vi "Network Read.vi"(8 "error in (no error)":errorcluster, 9 "Status_Cluster_in":T1={"simTime"=0.0, "simFrame"=0.0, "Connection Status"=enum."Disconnected", "Connection Command"=enum."Disconnect", "Last Error"=0, "Case selection"=enum."Connecting"}, 10 "RDB References in":T7, 11 "Settings":T4={"UDP Receiver"=refnum, "UDP Sender"=refnum, "Valid Packet"=FALSE, "TCP"=refnum, "Network Settings"={"IP adress"="127.0.0.1", "RDB"={"Protocol"=enum."UDP", "Tx Port"=48270, "Rx Port"=10, "Buffer Size"=204800, "Timeout"=10}, "SCP"={"Protocol"=enum."TCP", "Tx Port"=48191, "Rx Port"=48191, "Buffer Size"=204800, "Timeout"=10}}, "vclient"=path "", "paeseHandle"=0, "builderHandle"=0}) -> (0 "error out":errorcluster, 1 "Status_Cluster_out":T1={"simTime"=0.0, "simFrame"=0.0, "Connection Status"=enum."Disconnected", "Connection Command"=enum."Disconnect", "Last Error"=0, "Case selection"=enum."Connecting"}, 2 "RDB References out":T7, 3 "Settings":T4={"UDP Receiver"=refnum, "UDP Sender"=refnum, "Valid Packet"=FALSE, "TCP"=refnum, "Network Settings"={"IP adress"="127.0.0.1", "RDB"={"Protocol"=enum."UDP", "Tx Port"=48270, "Rx Port"=10, "Buffer Size"=204800, "Timeout"=10}, "SCP"={"Protocol"=enum."TCP", "Tx Port"=48191, "Rx Port"=48191, "Buffer Size"=204800, "Timeout"=10}}, "vclient"=path "", "paeseHandle"=0, "builderHandle"=0}, 5 "RDB Receive Reference.RDB Signals":dbl[](array[numeric]))   [LabVIEW 2023, in "Vires VTD Engine.lvlib"]
uses:
  Vires VTD Engine.lvlib
  RDB/RDB References.ctl
  DataContainer/DataContainer.lvclass
  Type/Settings.ctl
  Shared/Network Settings.ctl
  Shared/Protocol.ctl
  Type/Status_Cluster.ctl
  Type/ConnectionStatus.ctl
  Type/CaseSelection.ctl
  RDB/RDB.lvlib
  Shared/Vires VTD Shared.lvlib
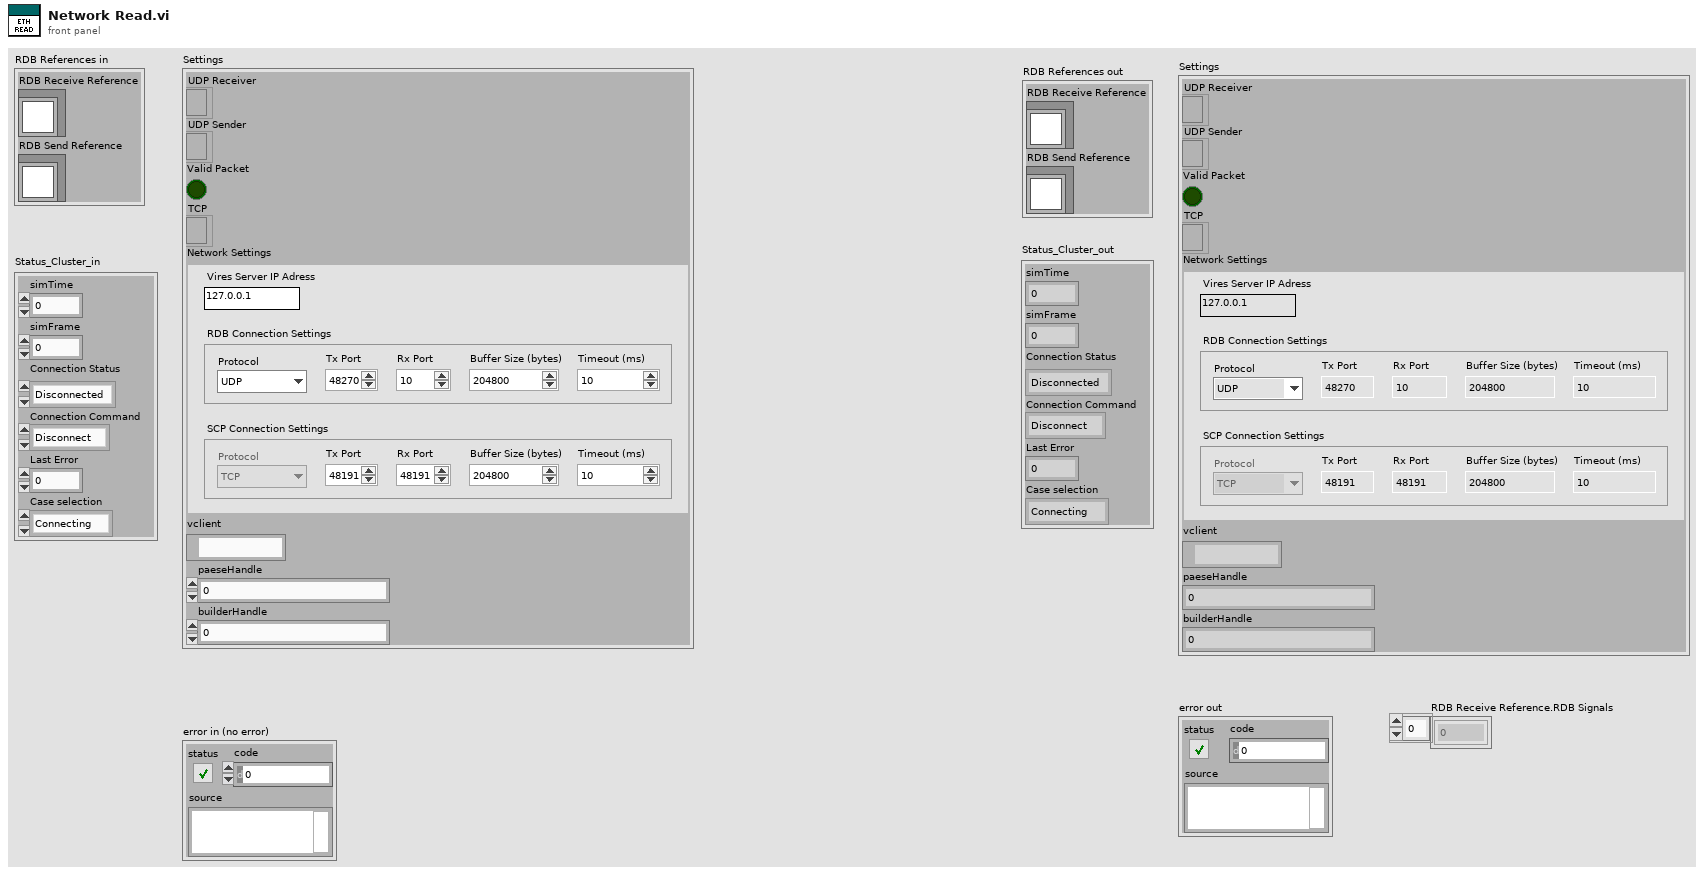
[diagram p1: front panel]
types:
  T1 = typedef "Vires VTD Engine.lvlib/Status_Cluster.ctl" = cluster{"simTime":dbl, "simFrame":dbl, "Connection Status":T2, "Connection Command":enum16{"Disconnect", "Connect"}, "Last Error":i32, "Case selection":T3}
  T2 = typedef "Vires VTD Engine.lvlib/ConnectionStatus.ctl" = enum16{"Disconnected", "Connected"}
  T3 = typedef "Vires VTD Engine.lvlib/CaseSelection.ctl" = enum32{"Idle", "Connecting", "Disconnecting", "Read/Write"}
  T4 = typedef "Vires VTD Engine.lvlib/Settings.ctl" = cluster{"UDP Receiver":refnum<k16>, "UDP Sender":refnum<k16>, "Valid Packet":bool, "TCP":refnum<k5>, "Network Settings":T5, "vclient":path, "paeseHandle":u64, "builderHandle":u64}
  T5 = typedef "Vires VTD Shared.lvlib/Network Settings.ctl" = cluster{"IP adress":string, "RDB":cluster{"Protocol":T6, "Tx Port":u16, "Rx Port":u16, "Buffer Size":i32, "Timeout":u16}, "SCP":cluster{"Protocol":T6, "Tx Port":u16, "Rx Port":u16, "Buffer Size":i32, "Timeout":u16}}
  T6 = typedef "Vires VTD Shared.lvlib/Protocol.ctl" = enum16{"UDP", "TCP"}
  T7 = typedef "RDB.lvlib/RDB References.ctl" = cluster{"RDB Receive Reference":refnum<class "DataContainer.lvclass">, "RDB Send Reference":refnum<class "DataContainer.lvclass">}
  T8 = enum16{"Standard", "Buffered", "CRLF", "Immediate"}
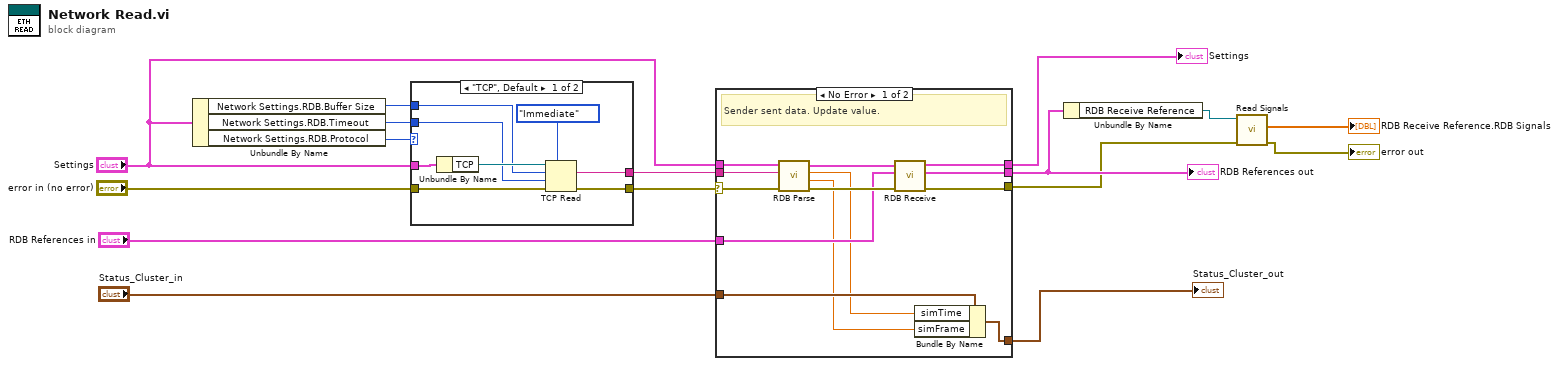
[diagram p0: block diagram]
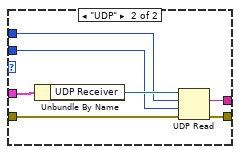
[diagram p2: hidden frame]
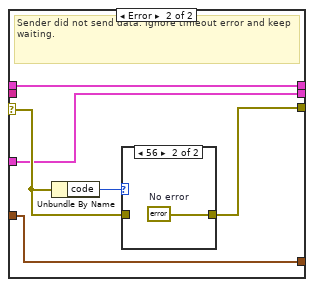
[diagram p3: hidden frame]
diagram:
  n1 = Unbundle By Name("Settings") -> ("Network Settings.RDB.Buffer Size"=w9:i32, "Network Settings.RDB.Timeout"=w10:u16, "Network Settings.RDB.Protocol"=w11:T6)
  n2 = case shown="\"TCP\", Default" w11 {
    tunnel: "error in (no error)" -> [w23 w31]
    tunnel: [w22 w30] -> w15
    tunnel: "Settings" -> [w24 w28]
    tunnel: [w21 w27] -> w5
    tunnel: w9 -> [w17 w26]
    tunnel: w10 -> [w18 w25]
    frame "TCP", Default {
      n3 = Unbundle By Name(w24) -> ("TCP"=w20:refnum<k5>)
      n4 = TCP Read(connection ID=w20, bytes to read=w17, error in (no error)=w23, 7:T8."Immediate" ("mode (standard)"), 9:w18) -> (data out=w21:string, error out=w22:errorcluster)  [unwired: 1 out]
    }
    frame "UDP" {
      n5 = Unbundle By Name(w28) -> ("UDP Receiver"=w29:refnum<k16>)
      n6 = UDP Read(connection ID=w29, max size (548)=w26, timeout ms (25000)=w25, 8:w31) -> (data out=w27:string, error out=w30:errorcluster)  [unwired: 3 out]
    }
  }
  n7 = case shown="No Error" w15 {
    selector: w15 -> [w44 w49]
    tunnel: [w41 w48] -> w2
    tunnel: "RDB References in" -> [w36 w47]
    tunnel: [w40 w47] -> w13
    tunnel: w5 -> [w42 _]
    tunnel: "Settings" -> [w39 w46]
    tunnel: [w37 w46] -> w12
    tunnel: "Status_Cluster_in" -> [w35 w45]
    tunnel: [w34 w45] -> w6
    frame No Error {
      # "Sender sent data. Update value."
      n8 = call "RDB Parse.vi"("error in (no error)"=w44, "RDB Message"=w42, "Settings"=w39) -> ("error out"=w43:errorcluster, "simFrame"=w32:dbl, "simTime"=w33:dbl, "Settings"=w38:T4)  [unwired: 5 in]
      n9 = call "RDB Receive.vi"("error in (no error)"=w43, "RDB Reference in"=w36, "Settings"=w38) -> ("error out"=w41:errorcluster, "RDB Reference out"=w40:T7, "Settings"=w37:T4)  [unwired: 6 in]
      n10 = Bundle By Name(cluster=w35, "simTime"=w33, "simFrame"=w32) -> (w34:T1)
    }
    frame Error {
      # "Sender did not send data. Ignore timeout error and keep waiting."
      n11 = Unbundle By Name(w49) -> ("code"=w50:i32)
      n12 = case shown="56" w50 {
        tunnel: w49 -> [w51 _]
        tunnel: [w51 w52] -> w48
        frame Default {
        }
        frame 56 {
          w52 = errorcluster {"status"=FALSE, "code"=0, "source"=""}  # No error
        }
      }
    }
  }
  "RDB References out" <- w13
  "Settings" <- w12
  "Status_Cluster_out" <- w6
  n13 = Unbundle By Name(w13) -> ("RDB Receive Reference"=w4:refnum<class "DataContainer.lvclass">)
  n14 = call-dynamic "Read Signals.vi"("error in (no error)"=w2, "DataContainer in"=w4) -> ("error out"=→"error out":errorcluster, "Signals"=→"RDB Receive Reference.RDB Signals":dbl[])  [unwired: 7 in, 1 out]
